vi "ZM-CP-publish.vi"(8 "error in (no error)":errorcluster, 10 "package":refnum<class "ZM-PC-package.lvclass">, 11 "ZM-CP-UDP-sender in":refnum<class "ZM-CP-UDP-sender.lvclass">) -> (0 "error out":errorcluster, 3 "ZM-CP-UDP-sender out":refnum<class "ZM-CP-UDP-sender.lvclass">)   [LabVIEW 2020, in "ZM-CP-UDP-udp_transport.lvlib" / "ZM-CP-UDP-sender.lvclass"]
doc: "The UDP sender's ZM-CP-publish: sends the package's JSON as one datagram to remoteAddress:remotePort (default 127.0.0.1:61557). Sending with no listener is silent (codes 66 and 56 cleared); every other error passes on. No Call Parent."
uses:
  ZM-CP-UDP-sender.lvclass
  common/ZM-PC-packages/ZM-PC-package/ZM-PC-package.lvclass
  ZM-CP-UDP-sender.lvclass/ZM-CP-UDP-sender.ctl
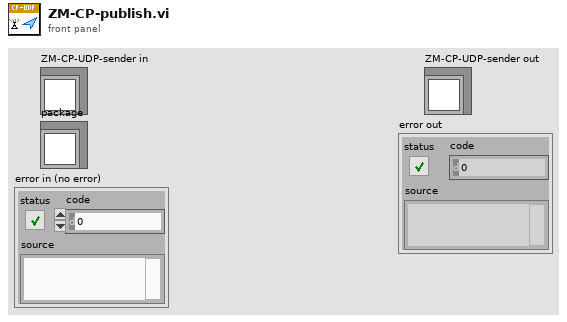
[diagram p1: front panel]
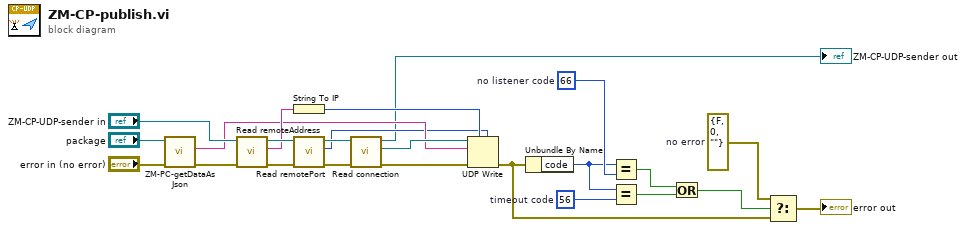
[diagram p0: block diagram]
diagram:
  w5 = errorcluster {"status"=FALSE, "code"=0, "source"=""}  # no error
  w8 = 56  # timeout code
  w10 = 66  # no listener code
  n1 = call-dynamic "ZM-PC-getDataAsJson.vi"("error in (no error)"="error in (no error)", "ZM-PC-package in"="package") -> ("error out"=w22:errorcluster, "json"=w14:string)  [unwired: 7 in, 1 out]
  n2 = call "Read remoteAddress.vi"("error in (no error)"=w22, "ZM-CP-UDP-sender in"="ZM-CP-UDP-sender in") -> ("error out"=w20:errorcluster, "remoteAddress"=w16:string, "ZM-CP-UDP-sender out"=w19:refnum<class "ZM-CP-UDP-sender.lvclass">)  [unwired: 7 in]
  n3 = String To IP(1:w16) -> (0:w12:u32)
  n4 = call "Read remotePort.vi"("error in (no error)"=w20, "ZM-CP-UDP-sender in"=w19) -> ("error out"=w18:errorcluster, "remotePort"=w11:u16, "ZM-CP-UDP-sender out"=w17:refnum<class "ZM-CP-UDP-sender.lvclass">)  [unwired: 7 in]
  n5 = call "Read connection.vi"("error in (no error)"=w18, "ZM-CP-UDP-sender in"=w17) -> ("error out"=w13:errorcluster, "connection"=w15:refnum<k16>, "ZM-CP-UDP-sender out"=→"ZM-CP-UDP-sender out":refnum<class "ZM-CP-UDP-sender.lvclass">)  [unwired: 7 in]
  n6 = UDP Write(address=w12, port or service name=w11, connection ID=w15, data in=w14, 8:w13) -> (error out=w3:errorcluster)  [unwired: 1 in, 1 out]
  n7 = Unbundle By Name(w3) -> ("code"=w9:i32)
  n8 = Equal?(x=w9, y=w10) -> (x = y?=w7:bool)
  n9 = Equal?(x=w9, y=w8) -> (x = y?=w6:bool)
  n10 = Or(x=w7, y=w6) -> (x .or. y?=w4:bool)
  n11 = Select(t=w5, s=w4, f=w3) -> (s? t:f=→"error out":errorcluster)
